vi "Utility - Set MC Listbox Icons.vi"(8 "error in":errorcluster, 9 "Icon Filenames":string[](array[string]), 10 "Symbol Indices":i32[](array[numeric]), 11 "MCListbox Refnum":refnum<vi>) -> (0 "error out":errorcluster)   [LabVIEW 2014]
doc: "::: VI Helpeks :::\nCopyright (c) 2000-2026 Konstantin Shifershteyn. All rights reserved."
panel:
  # "VI Helpeks\nCopyright (c) 2012-2026 Konstantin Shifershteyn"
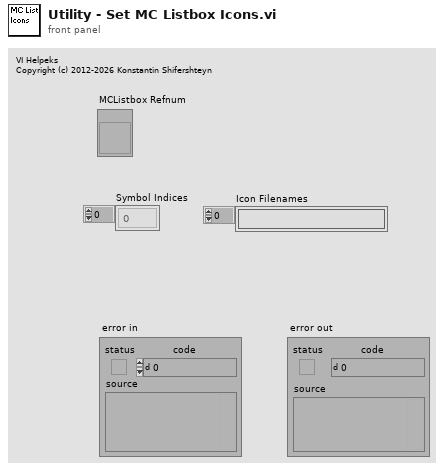
[diagram p1: front panel]
types:
  T1 = typedef "imagedata.ctl" = cluster{"image type":i32, "image depth":i32, "image":u8[], "mask":u8[], "colors":u32[], "Rectangle":cluster{"left":i16, "top":i16, "right":i16, "bottom":i16}}
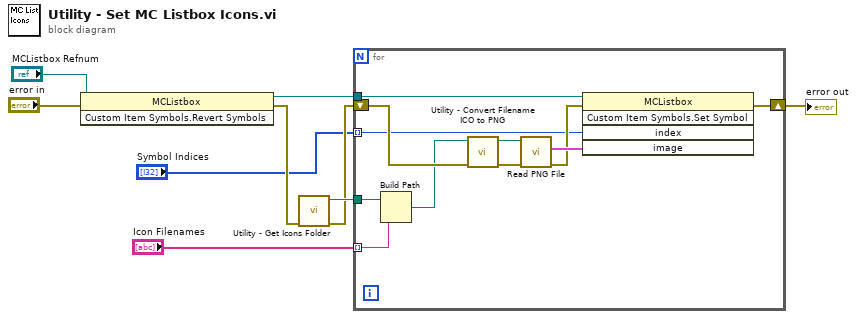
[diagram p0: block diagram]
diagram:
  n1 = invoke class="MCListbox" method="Custom Item Symbols.Revert Symbols"(reference="MCListbox Refnum", error in="error in") -> (reference out=w8:refnum<vi>, error out=w3:errorcluster)  [unwired: 1 in, 1 out]
  n2 = call "Utility - Get Icons Folder.vi"("error in"=w3) -> ("error out"=w4:errorcluster, "Icons Folder"=w5:path)  [unwired: 9 in]
  n3 = for {
    tunnel: w8 -> [w19]
    tunnel: w5 -> [w17]
    tunnel: "Icon Filenames" -> [w16] mode=indexing
    shift-right: [w15] -> w6
    shift-left: w4 -> [w14]
    tunnel: "Symbol Indices" -> [w12] mode=indexing
    n4 = Build Path(base path=w17, name or relative path=w16) -> (appended path=w10:path)
    n5 = call "Utility - Convert Filename ICO to PNG.vi"("Path"=w10) -> ("Path 2"=w11:path)  [unwired: 10 in]
    n6 = call <vilib>:"Read PNG File.vi"("error in (no error)"=w14, "path to PNG file"=w11) -> ("error out"=w13:errorcluster, "image data"=w18:T1)  [unwired: 7 in, 1 out]
    n7 = invoke class="MCListbox" method="Custom Item Symbols.Set Symbol"(reference=w19, error in=w13, "index"=w12, "image"=w18) -> (error out=w15:errorcluster)  [unwired: 1 in, 4 out]
  }
  "error out" <- w6
